vi "Add Error Description.vi"(9 "error in (no error)":errorcluster, 11 "error description":string) -> (1 "error out":errorcluster)   [LabVIEW 2019, in "Error Generation.lvlib"]
doc: "If error or warning add or replace an error description.\n- - -\nCopyright (c) 2023, Merecs Engineering GmbH"
uses:
  Error Generation.lvlib
panel:
  # "Connector Pane"
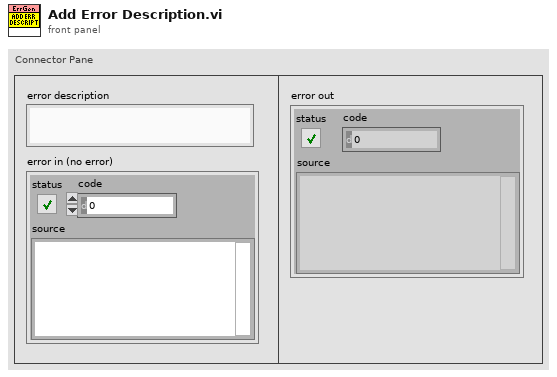
[diagram p1: front panel]
types:
  T1 = typedef "TagReturnType.ctl" = enum16{"No Tag", "<err>", "<append>"}
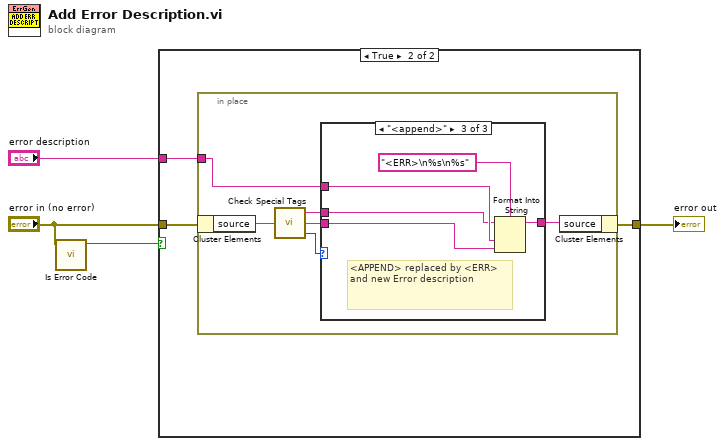
[diagram p0: block diagram]
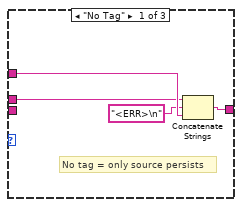
[diagram p3: hidden frame]
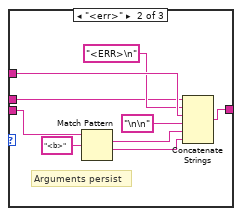
[diagram p4: hidden frame]
diagram:
  n1 = call "Is Error Code.vi"("error in (no error)"="error in (no error)") -> ("Code!=0"=w1:bool)  [unwired: 5 in, 1 out]
  n2 = case shown="True" w1 {
    tunnel: "error description" -> [_ w8]
    tunnel: [w5 w7] -> w3
    tunnel: "error in (no error)" -> [w5 w6]
    frame False {
    }
    frame True {
      n3 = in-place {
        in-place-border: w8 -> [w12]
        n4 = in-place-cluster #1(w6) -> ("source"=w10:string)
        n5 = call <vilib>:"Check Special Tags.vi"("source"=w10) -> ("Before Tag (source)"=w11:string, "After Tag (special data)"=w13:string, "Tag Found?"=w14:T1)
        n6 = case shown="\"<append>\"" w14 {
          tunnel: w13 -> [_ w23 w31]
          tunnel: w12 -> [w18 w27 w30]
          tunnel: [w17 w26 w29] -> w9
          tunnel: w11 -> [w15 w24 w28]
          frame "No Tag" {
            # "No tag = only source persists"
            n7 = Concatenate Strings(w15, "<ERR>\n" ("string"), w18) -> (w17:string)
          }
          frame "<err>" {
            # "Arguments persist"
            n8 = Match Pattern(string=w23, regular expression="<b>") -> (match substring=w22:string, after substring=w21:string)  [unwired: 1 in, 2 out]
            n9 = Concatenate Strings(w24, "<ERR>\n" ("string"), w27, "\n\n" ("string"), w22, w21) -> (w26:string)
          }
          frame "<append>" {
            # "<APPEND> replaced by <ERR> and new Error description"
            n10 = Format Into String(format string="<ERR>\n%s\n%s", initial string=w28, w30, w31) -> (resulting string=w29:string)  [unwired: 1 in, 1 out]
          }
        }
        n11 = in-place-cluster #1("source"=w9) -> (w7:errorcluster)
      }
    }
  }
  "error out" <- w3
